vi "打开引用.vi"(7 "引用":refnum<vi>, 8 "错误输入":errorcluster caption="错误输入（无错误）", 9 "CSM Name":string, 10 "VI":refnum<vi>) -> (0 "错误输出":errorcluster, 3 "VI输出":refnum<vi>)   [LabVIEW 2026, in "UI-Zolix.lvlib"]
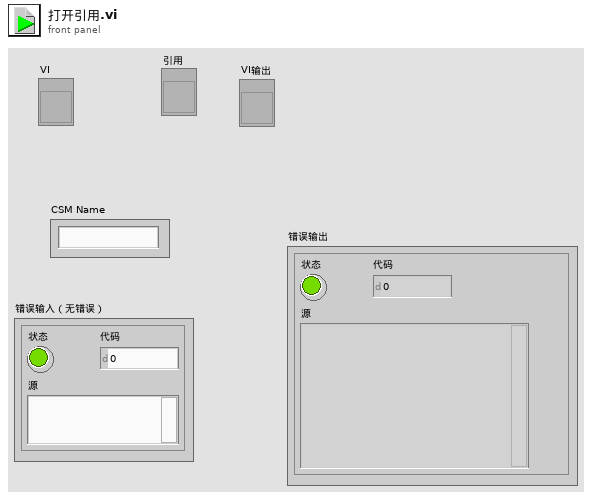
[diagram p1: front panel]
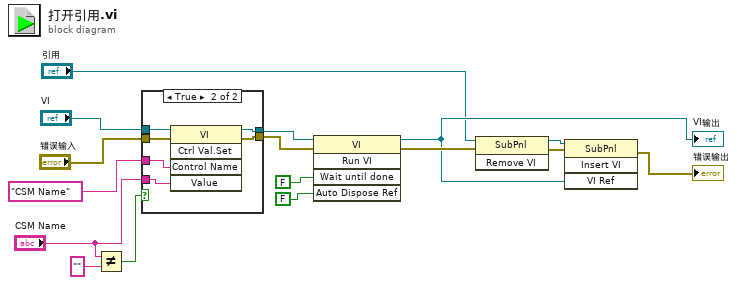
[diagram p0: block diagram]
diagram:
  n1 = Not Equal?(x="CSM Name", y="") -> (x != y?=w3:bool)
  n2 = case shown="True" w3 {
    tunnel: "VI" -> [w18 w24]
    tunnel: [w18 w23] -> w7
    tunnel: "CSM Name" ("控件名") -> [_ w22]
    tunnel: "CSM Name" -> [_ w21]
    tunnel: "错误输入" -> [w17 w20]
    tunnel: [w17 w19] -> w1
    frame False {
    }
    frame True {
      n3 = invoke class="VI" method="Ctrl Val.Set"(reference=w24, error in=w20, "Control Name"=w22, "Value"=w21) -> (reference out=w23:refnum<vi>, error out=w19:errorcluster)  [unwired: 1 in, 3 out]
    }
  }
  n4 = invoke on="Invoke Node" class="VI" method="Run VI"(reference=w7, error in=w1, "Wait until done"=FALSE ("Wait Until Done"), "Auto Dispose Ref"=FALSE ("Auto Dispose Reference")) -> (reference out=w13:refnum<vi>, error out=w14:errorcluster)  [unwired: 1 in, 3 out]
  "VI输出" <- w13
  n5 = invoke class="SubPnl" method="Remove VI"(reference="引用", error in=w14) -> (reference out=w15:refnum<vi>, error out=w16:errorcluster)  [unwired: 1 in, 1 out]
  n6 = invoke class="SubPnl" method="Insert VI"(reference=w15, error in=w16, "VI Ref"=w13) -> (error out=→"错误输出":errorcluster)  [unwired: 1 in, 3 out]
